vi "1.Test_Sequence.vi"() -> ()   [LabVIEW 2021]
uses:
  Control/Test_Case.ctl
  Control/Set_Get.ctl
  HI-POT_Driver/Hi-pot_Driver.ctl
  Control/Ini.ctl
panel:
  in  "error in (no error) 3":errorcluster
  out "path":path
  out "?":string
  out "Serial Number":string
  in  "error in (no error)":errorcluster
  out "Color Box":u32(colorbox)
  out "BARCODE":string
  out "Expected 2":string
  out "Measured2":string
  out "Applied 2":string
  out "Measured":string
  out "Applied":string
  out "Expected":string
  in  "Start Button 2":bool
  in  "Exit 2":bool
  in  "Multicolumn Listbox":i32(listbox)
  # "PROFILE"
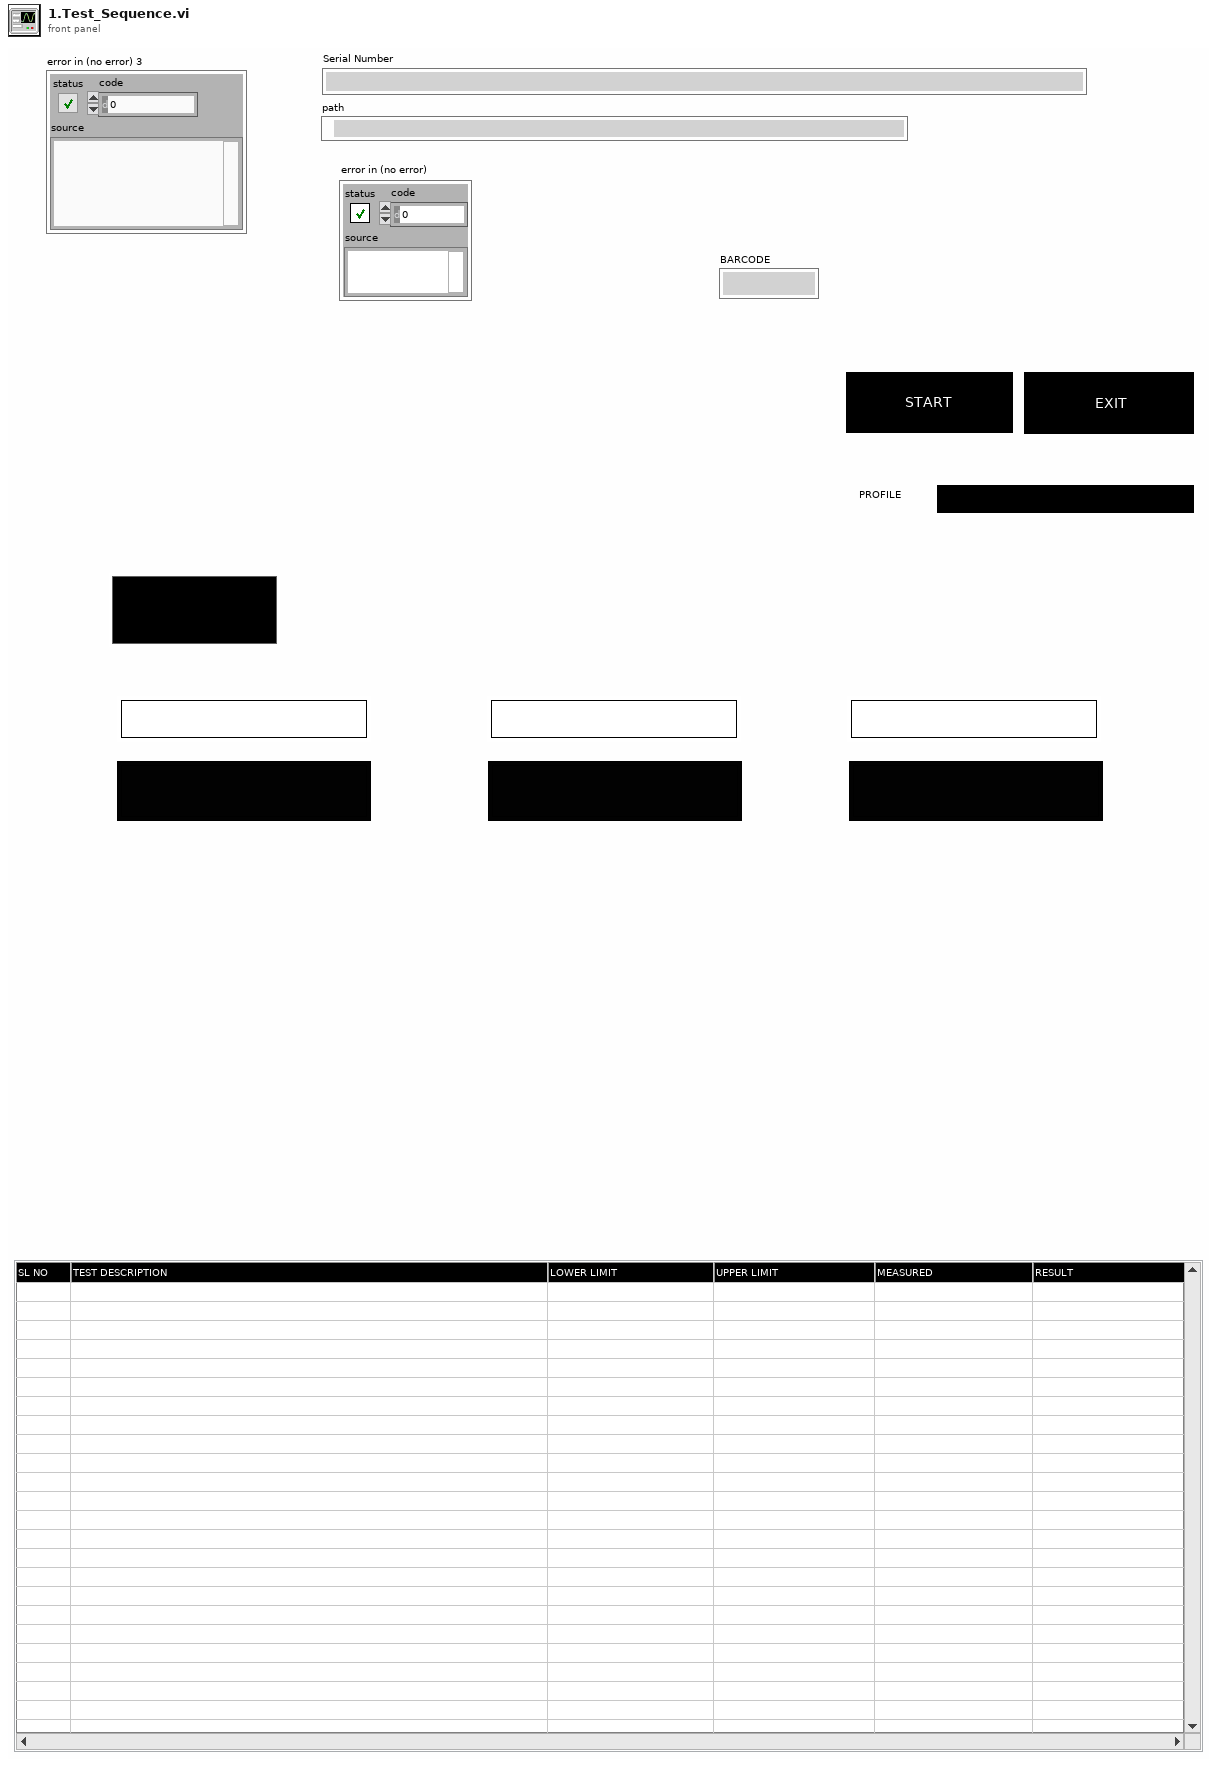
[diagram p1: front panel]
types:
  T1 = typedef "Set_Get.ctl" = enum16{"Set", "Get"}
  T2 = typedef "Test_Case.ctl" = enum16{"Init", "Idle State", "Scan Barcode", "Power ON and Setup", "Measuring the leakage current", "Result", "Report", "Exit"}
  T3 = typedef "Ini.ctl" = enum16{"Write", "Read"}
  T4 = typedef "Hi-pot_Driver.ctl" = enum16{"Init ", "Set UP DCW", "Set UP ACW", "Set UP IR", "Read", "Clear", "Close"}
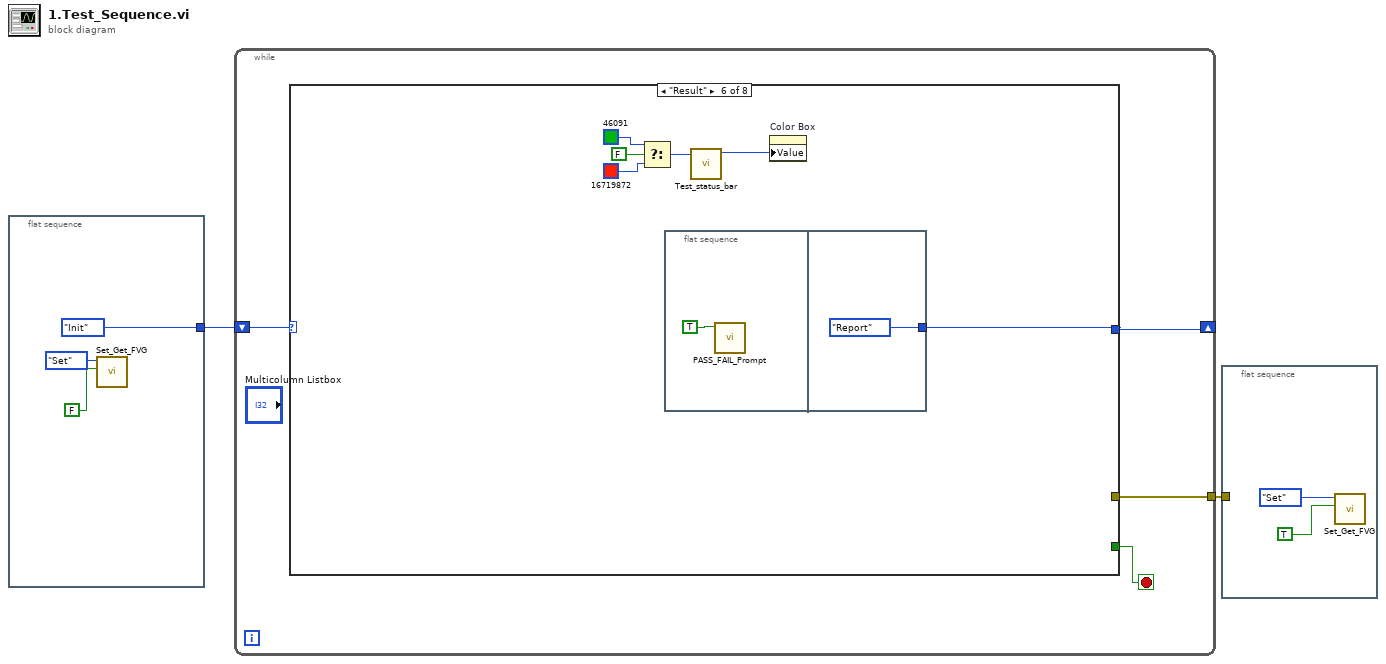
[diagram p0: block diagram]
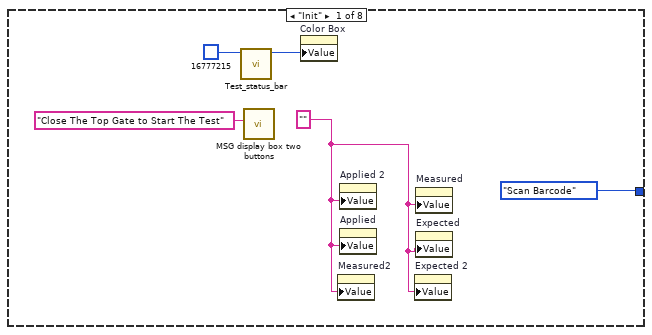
[diagram p2: hidden frame]
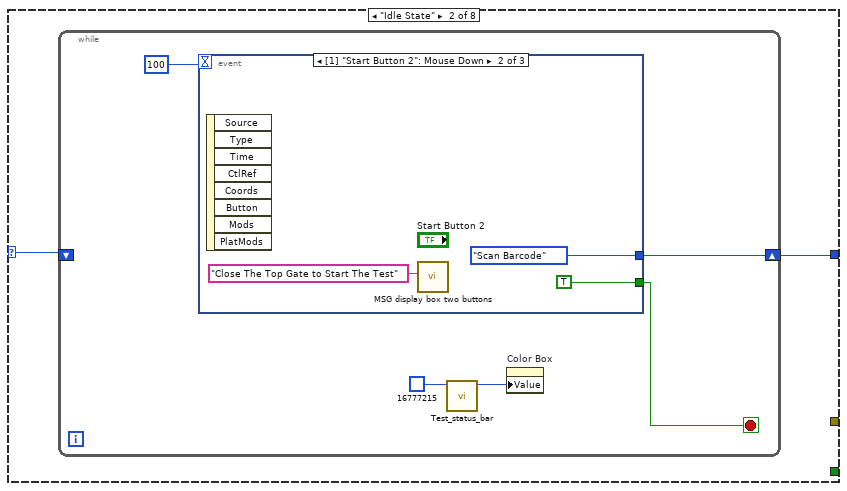
[diagram p3: hidden frame]
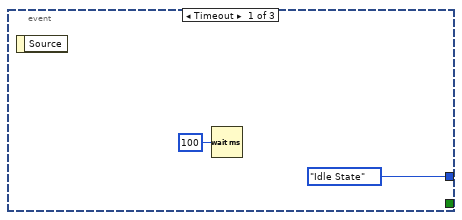
[diagram p4: hidden frame]
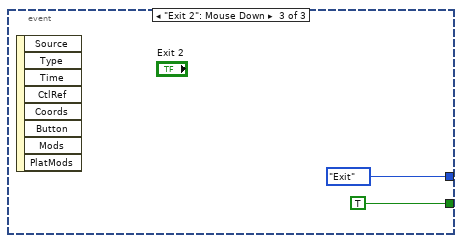
[diagram p5: hidden frame]
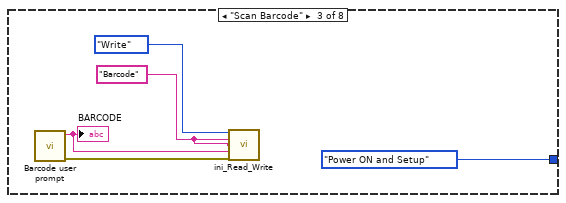
[diagram p6: hidden frame]
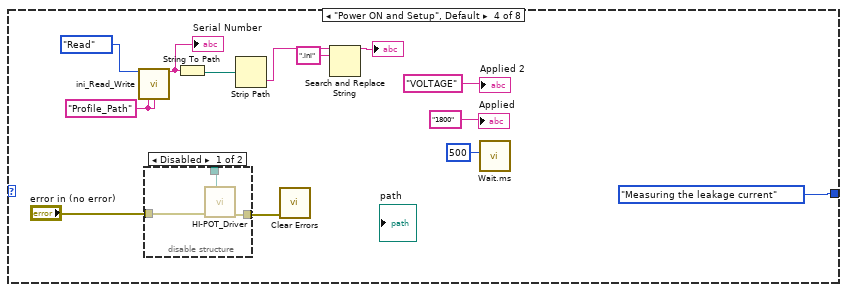
[diagram p7: hidden frame]
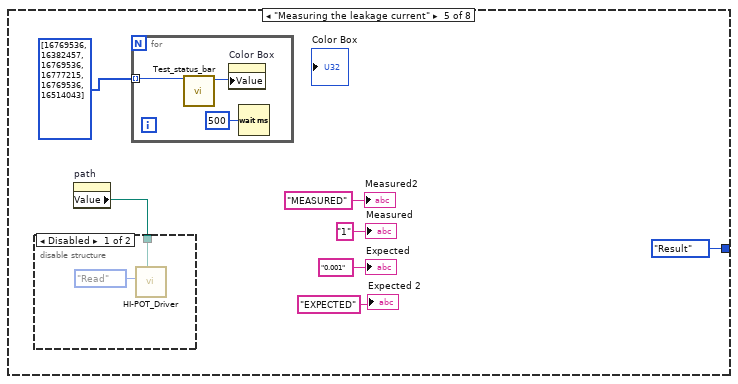
[diagram p9: hidden frame]
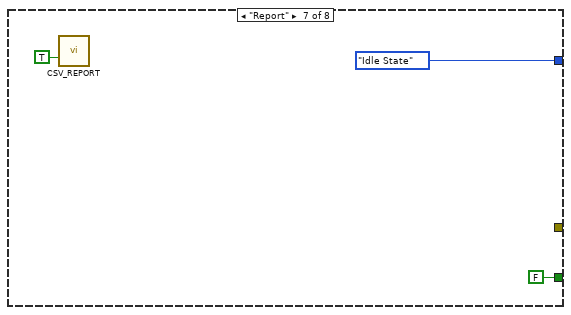
[diagram p11: hidden frame]
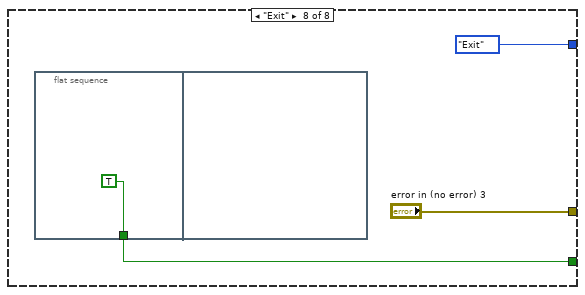
[diagram p12: hidden frame]
diagram:
  n1 = flat-sequence {
    tunnel: [Test_Case."Init"] -> w2
    frame #0 {
      n2 = call "Set_Get_FVG.vi"("Message"=FALSE ("Set"), "Enum"=Set_Get."Set") -> ()  [unwired: 7 in, 3 out]
    }
  }
  n3 = while {
    shift-right: [w7] -> _
    shift-left: w2 -> [w8]
    tunnel: [w6] -> w1
    stop <- w9 stop-if-true
    n4 = case shown="\"Result\"" w8 {
      selector: w8 -> [_ w15 _ _ _ _ _ _]
      tunnel: [_ _ _ _ _ _ FALSE w74] -> w9
      tunnel: [Test_Case."Scan Barcode" w16 Test_Case."Power ON and Setup" Test_Case."Measuring the leakage current" Test_Case."Result" w67 Test_Case."Idle State" Test_Case."Exit"] -> w7
      tunnel: [_ _ _ _ _ _ _ "error in (no error) 3"] -> w6
      frame "Init" {
        w12 = "" ("Measured2")
        n5 = call "Test_status_bar.vi"("Color Box  2"=u32 16777215 ("Color Box 3")) -> ("Color Box"=w10:u32)  [unwired: 10 in]
        n6 = call "MSG display box two buttons.vi"("input string"="Close The Top Gate to Start The Test") -> ()  [unwired: 8 in, 3 out]
        n7 = property on="Color Box" class="ColBox"("Value"=w10) -> ()  [unwired: 2 in, 2 out]
        n8 = property on="Measured2" class="Str"("Value"=w12) -> ()  [unwired: 2 in, 2 out]
        n9 = property on="Applied 2" class="Str"("Value"=w12) -> ()  [unwired: 2 in, 2 out]
        n10 = property on="Applied" class="Str"("Value"=w12) -> ()  [unwired: 2 in, 2 out]
        n11 = property on="Expected 2" class="Str"("Value"=w12) -> ()  [unwired: 2 in, 2 out]
        n12 = property on="Measured" class="Str"("Value"=w12) -> ()  [unwired: 2 in, 2 out]
        n13 = property on="Expected" class="Str"("Value"=w12) -> ()  [unwired: 2 in, 2 out]
      }
      frame "Idle State" {
        n14 = while {
          shift-right: [w20] -> w16
          shift-left: w15 -> [_]
          stop <- w21 stop-if-true
          n15 = event shown="[1] \"Start Button 2\": Mouse Down" {
            selector: _ -> [_ _ _]
            dyn-events: _ -> [_ _ _]
            timeout: 100 -> [_ _ _]
            tunnel: [_ TRUE TRUE] -> w21
            tunnel: [Test_Case."Idle State" Test_Case."Scan Barcode" Test_Case."Exit"] -> w20
            event Timeout {
              n16 = event-data() -> ()  [unwired: 1 in, 1 out]
              n17 = Wait (ms)(milliseconds to wait=u32 100) -> ()  [unwired: 1 out]
            }
            event "Start Button 2": Mouse Down {
              n18 = event-data() -> ()  [unwired: 1 in, 8 out]
              n19 = call "MSG display box two buttons.vi"("input string"="Close The Top Gate to Start The Test") -> ()  [unwired: 8 in, 3 out]
            }
            event "Exit 2": Mouse Down {
              n20 = event-data() -> ()  [unwired: 1 in, 8 out]
            }
          }
          n21 = call "Test_status_bar.vi"("Color Box  2"=u32 16777215 ("Color Box 3")) -> ("Color Box"=w17:u32)  [unwired: 10 in]
          n22 = property on="Color Box" class="ColBox"("Value"=w17) -> ()  [unwired: 2 in, 2 out]
        }
      }
      frame "Scan Barcode" {
        w30 = "Barcode" ("Write Section")
        n23 = call "Barcode user prompt.vi"() -> ("error out"=w31:errorcluster, "BARCODE"=w29:string)  [unwired: 9 in, 1 out]
        "BARCODE" <- w29
        n24 = call "ini_Read_Write.vi"(0:Ini."Write", "Write Section"=w30, "Write key"=w30, "Write"=w29, "error in (no error) 2"=w31) -> ()  [unwired: 9 in, 2 out]
      }
      frame "Power ON and Setup", Default {
        w39 = "Profile_Path" ("Read Section")
        n25 = call "ini_Read_Write.vi"(0:Ini."Read", "Read Section"=w39, "Read Key"=w39) -> ("value"=w38:string)  [unwired: 11 in, 1 out]
        "Serial Number" <- w38
        n26 = disable-structure shown="Disabled" {
          disable-tunnel: "error in (no error)" -> [w49 _]
          disable-tunnel: [w48 _] -> w43
          disable-tunnel: _ -> [w47 _]
          frame Disabled {
            n27 = call "HI-POT_Driver.vi"("configuration file path"=w47, "error in (no error)"=w49) -> ("error out"=w48:errorcluster)  [unwired: 7 in, 2 out]
          }
          frame Enabled {
          }
        }
        n28 = String To Path(string=w38) -> (path=w37:path)
        n29 = Strip Path(path=w37) -> (name=w36:string)  [unwired: 1 out]
        n30 = call <vilib>:"Clear Errors.vi"("error in (no error)"=w43) -> ()  [unwired: 5 in, 2 out]
        n31 = Search and Replace String(input string=w36, search string=".ini") -> (result string=→"?":string)  [unwired: 6 in, 3 out]
        n32 = call "Wait.ms.vi"("milliseconds to wait"=u32 500) -> ()  [unwired: 10 in, 1 out]
        "Applied" <- "1800" ("String Indicator 4")
        "Applied 2" <- "VOLTAGE" ("String Indicator 6")
      }
      frame "Measuring the leakage current" {
        n33 = property on="path" class="Path"() -> ("Value"=w50:path)  [unwired: 2 in, 2 out]
        n34 = disable-structure shown="Disabled" {
          disable-tunnel: w50 -> [w57 _]
          frame Disabled {
            n35 = call "HI-POT_Driver.vi"("configuration file path"=w57, 10:Hi-pot_Driver."Read") -> ()  [unwired: 7 in, 3 out]
          }
          frame Enabled {
          }
        }
        n36 = for {
          tunnel: u32[] [16769536, 16382457, 16769536, 16777215, 16769536, 16514043] -> [w60] mode=indexing
          n37 = call "Test_status_bar.vi"("Color Box  2"=w60) -> ("Color Box"=w61:u32)  [unwired: 10 in]
          n38 = property on="Color Box" class="ColBox"("Value"=w61) -> ()  [unwired: 2 in, 2 out]
          n39 = Wait (ms)(milliseconds to wait=u32 500) -> ()  [unwired: 1 out]
        }
        "Measured" <- "1" ("Measured")
        "Measured2" <- "MEASURED" ("String Indicator 6")
        "Expected" <- "0.001" ("Expected")
        "Expected 2" <- "EXPECTED" ("Expected 2")
      }
      frame "Result" {
        n40 = Select(t=u32 46091 ("Color Box 3"), s=FALSE, f=u32 16719872 ("Color Box 3")) -> (s? t:f=w64:u32)
        n41 = flat-sequence {
          tunnel: [Test_Case."Report"] -> w67
          frame #0 {
            n42 = call "PASS_FAIL_Prompt.vi"("Result"=TRUE) -> ()  [unwired: 11 in]
          }
          frame #1 {
          }
        }
        n43 = call "Test_status_bar.vi"("Color Box  2"=w64) -> ("Color Box"=w66:u32)  [unwired: 10 in]
        n44 = property on="Color Box" class="ColBox"("Value"=w66) -> ()  [unwired: 2 in, 2 out]
      }
      frame "Report" {
        n45 = call "CSV_REPORT.vi"("Result"=TRUE) -> ()  [unwired: 27 in]
      }
      frame "Exit" {
        n46 = flat-sequence {
          tunnel: [TRUE] -> w74
          frame #0 {
          }
          frame #1 {
          }
        }
      }
    }
  }
  n47 = flat-sequence {
    tunnel: w1 -> [_]
    frame #0 {
      n48 = call "Set_Get_FVG.vi"("Message"=TRUE ("Set"), "Enum"=Set_Get."Set") -> ()  [unwired: 7 in, 3 out]
    }
  }
